vi "calc_curvarture.vi"(9 "Near Point":dbl, 10 "mid_far_edge":i32, 11 "mid_near_edge":i32) -> (3 "kappa":dbl)   [LabVIEW 2024]
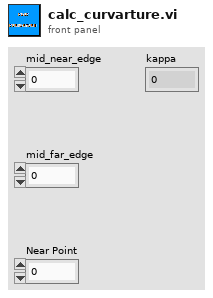
[diagram p1: front panel]
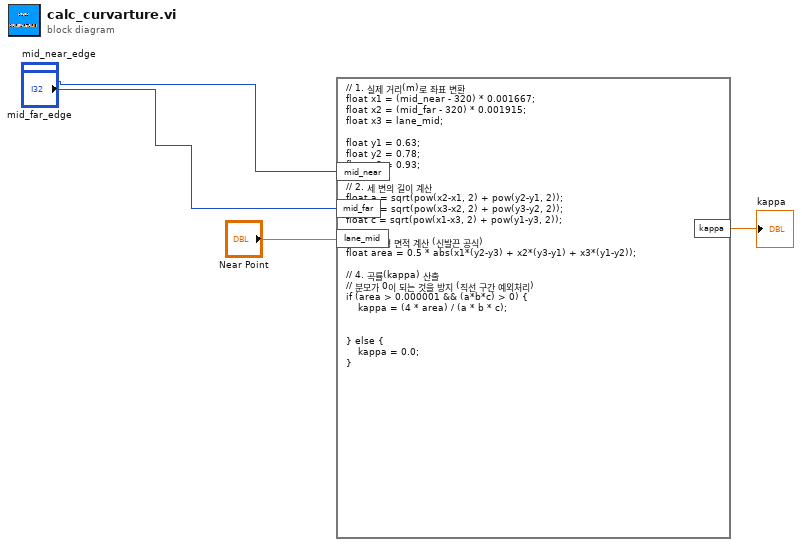
[diagram p0: block diagram]
diagram:
  n1 = formula code="// 1. 실제 거리(m)로 좌표 변환\nfloat x1 = (mid_near - 320) * 0.001667;\nfloat x2 = (mid_far - 320) * 0.001915;\nfloat x3 = lane_mid;\n\nfloat y1 = 0.63;\nfloat y2 = 0.78;\nfloat y3 = 0.93;\n\n// 2. 세 변의 길이 계산\nfloat a = sqrt(pow(x2-x1, 2) + pow(y2-y1, 2));\nfloat b = sqrt(pow(x3-x2, 2) + pow(y3-y2, 2));\nfloat c = sqrt(pow(x1-x3, 2) + pow(y1-y3, 2));\n\n// 3. 삼각형 면적 계산 (신발끈 공식)\nfloat area = 0.5 * abs(x1*(y2-y3) + x2*(y3-y1) + x3*(y1-y2));\n\n// 4. 곡률(kappa) 산출\n// 분모가 0이 되는 것을 방지 (직선 구간 예외처리)\nif (area > 0.000001 && (a*b*c) > 0) {\n    kappa = (4 * area) / (a * b * c);\n    \n    \n} else {\n    kappa = 0.0;\n}"("mid_near"="mid_near_edge", "mid_far"="mid_far_edge", "lane_mid"="Near Point") -> ("kappa"=→"kappa":dbl)
